vi "CSM-Logger-Thread(Event).vi"(4 "Log Limit":T1={"file size (in bytes)"=10000000, "file num"=2} {"file size (in bytes)" format="%.0p"}, 6 "Exit When All Module Exist? (F)":bool, 7 "Format String":string="%<%Y/%m/%d %H:%M:%S%3u>T", 8 "error in (no error)":errorcluster, 9 "WatchDogQ":refnum<queue>, 10 "GlobalLogFilter.lvclass":refnum<class "LogFilter.lvclass">, 11 "File Path (Use Dialog)":path) -> (0 "error out":errorcluster)   [LabVIEW 2017, in "CSM File Logger.lvlib"]
doc: "The thread VI originally used in the CSM - Start File Logger VI. This VI is now deprecated. Use the CSM-Logger-Thread VI.\n\n\n> [!NOTE] <b>CSM File Logger Implementation Principle</b>\n>\n> The CSM File Logger retrieves all execution records in the application via the CSM Global Log API and saves them to a specified text file for later analysis and error localization. The file format is a text file with the suffix `.csmlog`, which can be opened using text editing query tools such as Notepad."
uses:
  CSM File Logger.lvlib
  CSM File Logger Limit.ctl
  _Support/GlobalEvent/LogFilter/LogFilter.lvclass
  _Support/Typedef/_CSM_List Module Scope.ctl
  _Support/Typedef/_CSM_GlobalLog_MSG.ctl
  _Support/Typedef/_CSM_Response Source Message.ctl
  _Support/Typedef/_CSM_GlobalLog_MSG_TYPE.ctl
  Utility/_support/Periodic String Filter Level.ctl
  _Support/GlobalEvent/GEvt-Generate with Rule Check.vi
  AdvanceAPI/CSM - Convert Error to Argument.vi
  _Support/GlobalEvent/Cache-GEvt Filter Object.vi
  _Support/GlobalEvent/Cache-GEvt Refs.vi
  AdvanceAPI/CSM - Make String Arguments Safe.vi
  _Support/GlobalEvent/GEvt-Convert Filter Rules - v1.2.vi
  _Support/ChangeFlag/FlagInstance-GEvt Filter.vi
  _Support/ChangeFlag/FlagInstance-GEvt Refs.vi
  AdvanceAPI/CSM - Keywords.vi
  _Support/ChangeFlag/ChangeFlag-Read.vi
  _Support/GlobalEvent/LogFilter/SettingVIs/Set Periodic Log Filter.vi
  _Support/GlobalEvent/LogFilter/SettingVIs/Set CSM UserLog Filter.vi
  _Support/GlobalEvent/LogFilter/SettingVIs/Set CSM Broadcast Filter.vi
  _Support/GlobalEvent/LogFilter/SettingVIs/Set CSM StateType Filter.vi
  _Support/GlobalEvent/LogFilter/SettingVIs/Set Global StateType Filter.vi
  _Support/GlobalEvent/LogFilter/SettingVIs/Set CSM State Filter.vi
  _Support/GlobalEvent/LogFilter/SettingVIs/Set CSM LogType Filter.vi
  _Support/GlobalEvent/LogFilter/SettingVIs/Set Global UserLog Filter.vi
  _Support/GlobalEvent/LogFilter/SettingVIs/Set Global Broadcast Filter.vi
  _Support/GlobalEvent/LogFilter/SettingVIs/Set Global State Filter.vi
  _Support/GlobalEvent/LogFilter/SettingVIs/Set Global LogType Filter.vi
  _Support/GlobalEvent/LogFilter/SettingVIs/Set Global CSM Filter.vi
  _Support/GlobalEvent/FGV-GEvt Filter Rules(lvlibp).vi
  _Support/ChangeFlag/ChangeFlagDB.vi
  _Support/GlobalEvent/GEvt-Valid Subscribers.vi
  _Support/GlobalEvent/FGV-GlobalEventQueues(lvlibp).vi
  _Support/GlobalEvent/FGV-GlobalEventRef(lvlibp).vi
  Communicable State Machine.lvlib
panel:
  out "size (in bytes)":i64
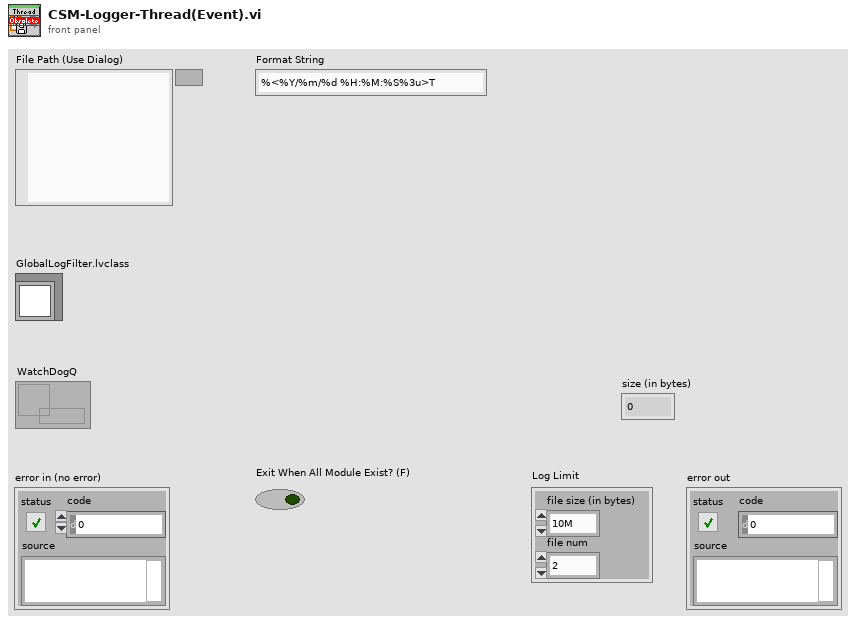
[diagram p1: front panel]
types:
  T1 = typedef "CSM File Logger.lvlib/CSM File Logger Limit.ctl" = cluster{"file size (in bytes)":i64, "file num":i32}
  T2 = typedef "Communicable State Machine.lvlib/_CSM_GlobalLog Filter Rules - v1.2.ctl" = cluster{"Global":cluster{"CSM":string[], "LogType":T3[], "State":string[], "StateType":T4[], "Broadcast":string[], "UserLog":string[]}, "CSM":cluster{"LogType":cluster{"CSM":string, "LogType":T3}[], "State":cluster{"CSM":string, "State":string}[], "StateType":cluster{"CSM":string, "LogType":T4}[], "Broadcast":cluster{"CSM":string, "Broadcast":string}[], "UserLog":cluster{"CSM":string, "UserLog":string}[]}, "PeriodicMessageFilter":cluster{"Enable":bool, "Threshold(#/s)":dbl, "CheckPeriod(s)":dbl}}
  T3 = typedef "Communicable State Machine.lvlib/_CSM_GlobalLog_MSG_TYPE.ctl" = enum16{"User Log", "State Change", "Status", "Interrupt", "Register", "Unregister", "Error Log", "Module Created", "Module Destroyed", "Async Message", "No-Rep Async Message", "Sync Message", "AsyncMsg Complete", "SyncMsg Complete"}
  T4 = typedef "Communicable State Machine.lvlib/_CSM_GlobalLog_STATE_TYPE.ctl" = enum16{"State - Internal State", "State - External Message", "State - Response", "State - Complete"}
  T5 = cluster{"Queue":path[], "folder":path, "name":string, "index":i32, "Log Limit":T1}
  T6 = typedef "Communicable State Machine.lvlib/_CSM_List Module Scope.ctl" = enum16{"Normal", "System Only", "All"}
  T7 = typedef "Communicable State Machine.lvlib/Periodic String Filter Level.ctl" = enum16{"normal", "L1", "L2", "L3", "L4"}
  T8 = typedef "Communicable State Machine.lvlib/_CSM_GlobalLog_MSG.ctl" = cluster{"Name (\"\" to Use UUID)":string, "Current State":string, "Arguments":string, "Source Message":T9, "Source Module":string, "Complete(T)/Start(F)":bool, "LogType":T3, "Time Stamp":timestamp}
  T9 = typedef "Communicable State Machine.lvlib/_CSM_Response Source Message.ctl" = cluster{"‘State":string, "’Arguments":string, "’Error":errorcluster}
  T10 = enum16{"open", "replace", "create", "open or create", "replace or create", "replace or create with confirmation"}
  T11 = cluster{"Major":u16, "Minor":u16, "Fix":u16, "Build":u16}
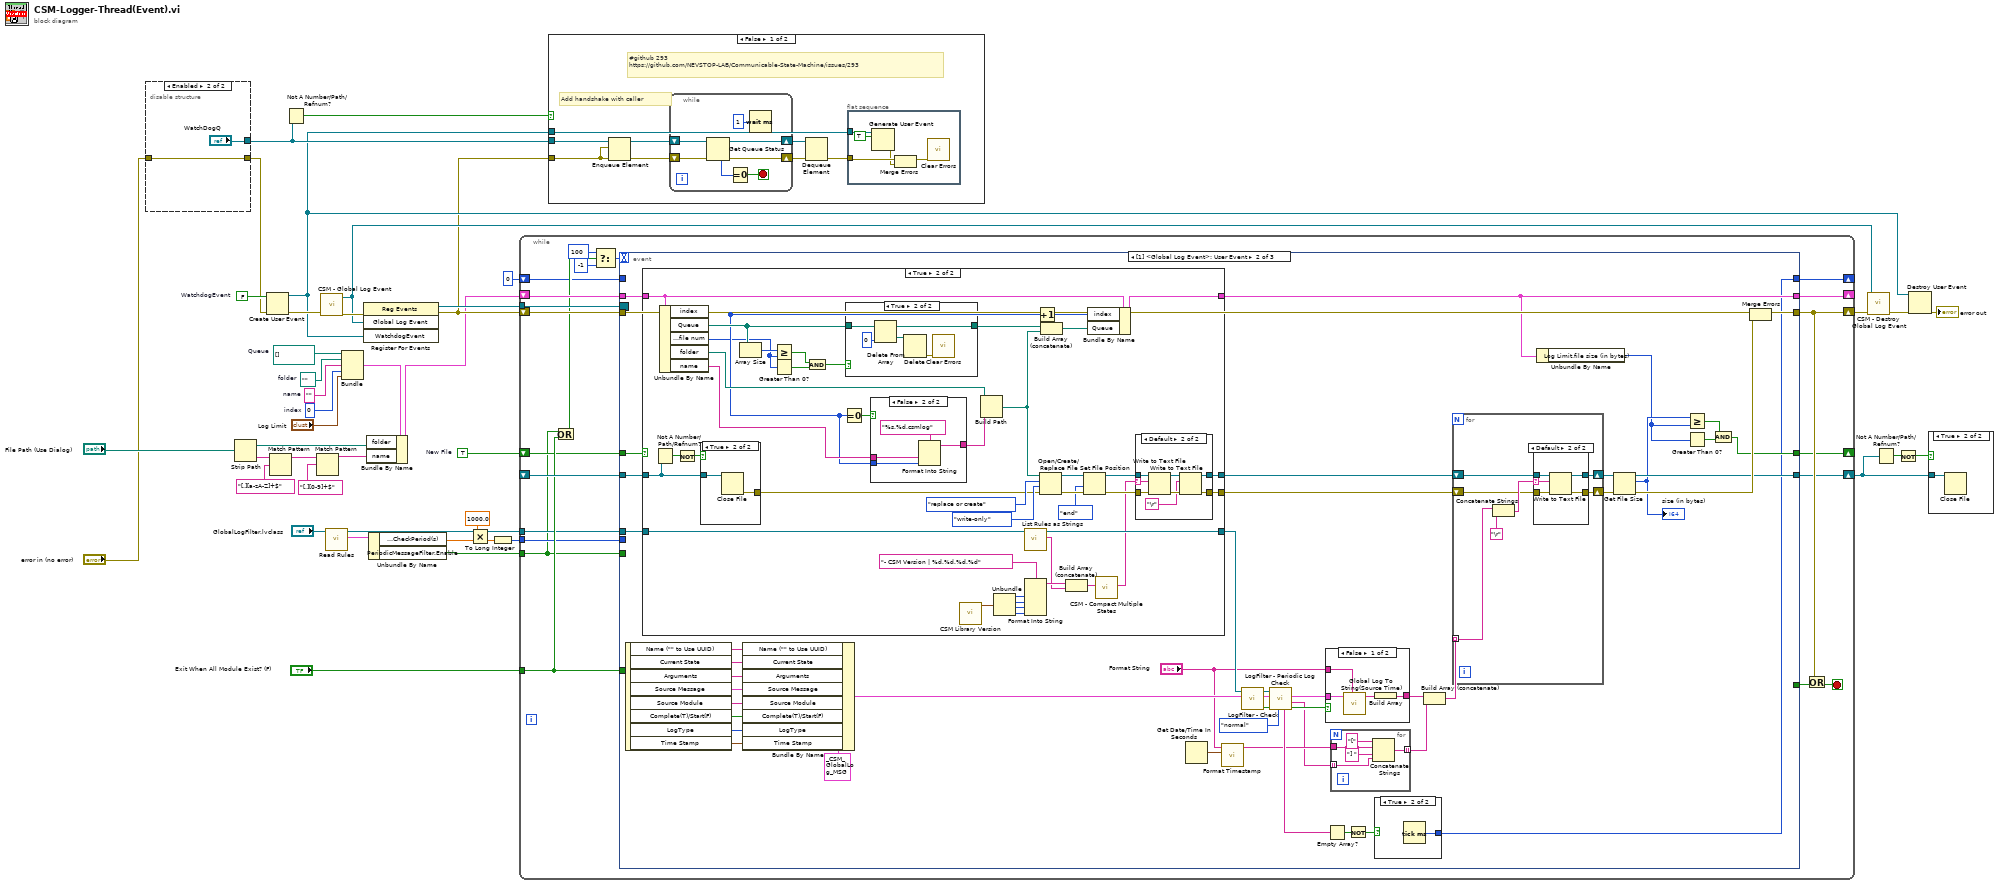
[diagram p0: block diagram]
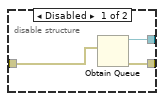
[diagram p2: hidden frame]
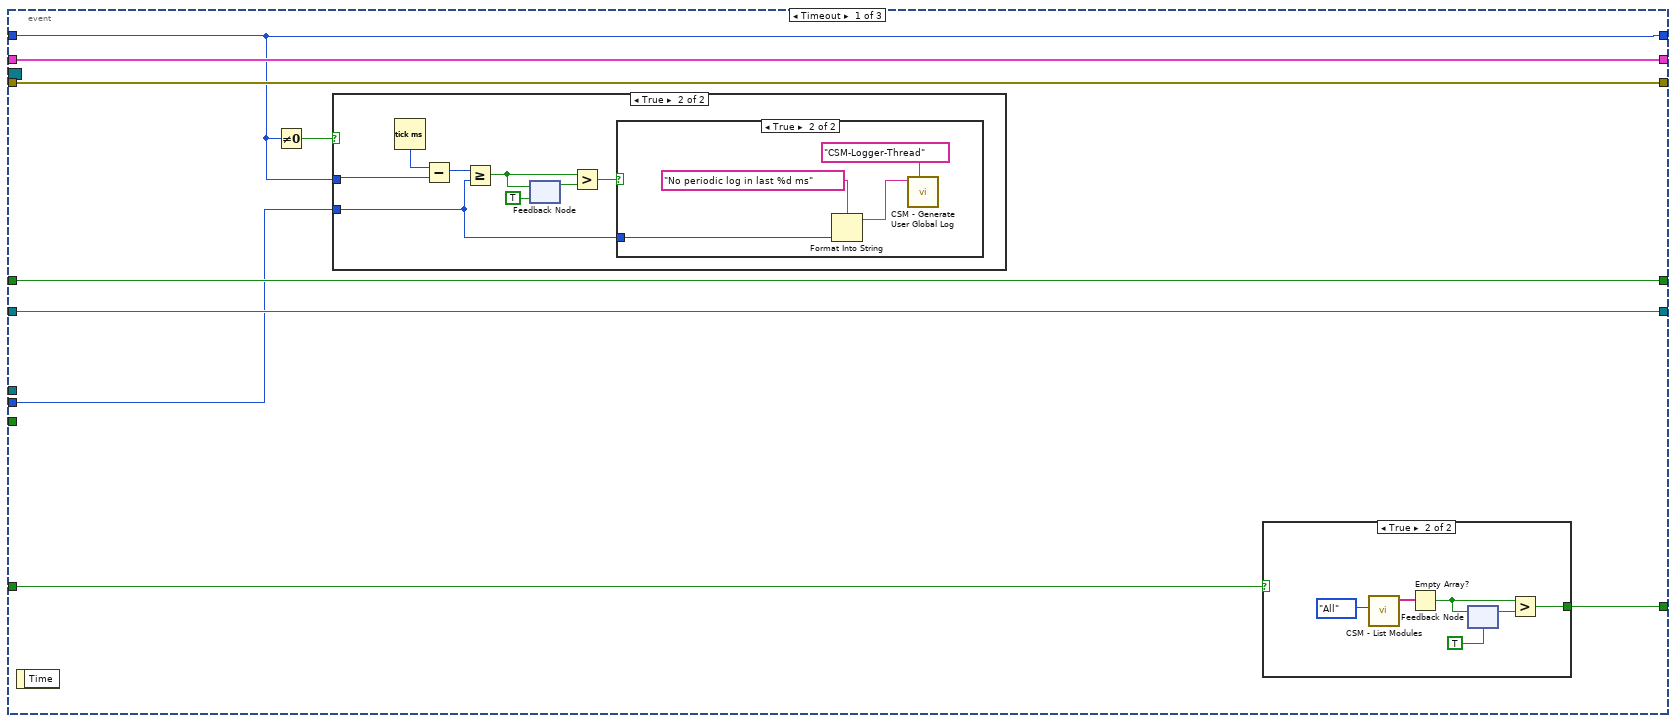
[diagram p5: hidden frame]
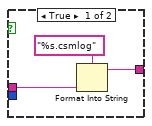
[diagram p14: hidden frame]
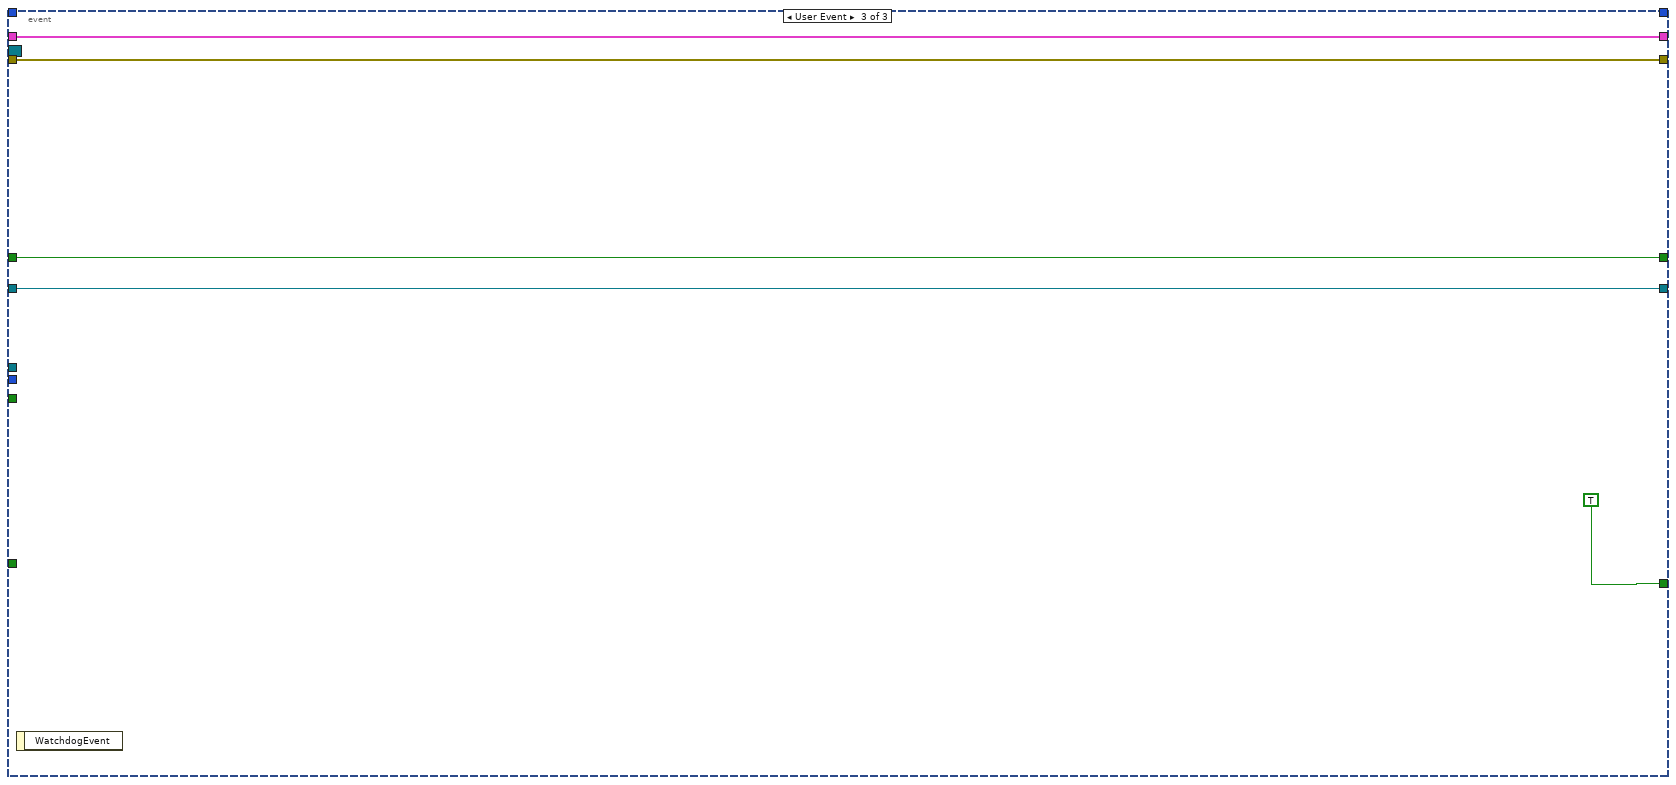
[diagram p17: hidden frame]
diagram:
  w19 = ""  # name
  w22 = 0  # index
  w23 = path ""  # folder
  w24 = path[] []  # Queue
  w27 = TRUE  # New File
  w36 = FALSE  # WatchdogEvent
  n1 = disable-structure shown="Enabled" {
    disable-tunnel: [w43 "WatchDogQ"] -> w38
    disable-tunnel: [w45 w46] -> w26
    disable-tunnel: "error in (no error)" -> [w44 w46]
    frame Disabled {
      n2 = Obtain Queue(element data type=w44) -> (queue out=w43:refnum<queue>, error out=w45:errorcluster)  [unwired: 4 in, 1 out]
    }
    frame Enabled {
    }
  }
  n3 = Strip Path(path="File Path (Use Dialog)") -> (stripped path=w12:path, name=w18:string)
  n4 = Create User Event(user event datatype=w36, error in=w26) -> (user event=w33:refnum<user-event>, error out=w35:errorcluster)
  n5 = Match Pattern(string=w18, regular expression="[.][a-zA-Z]+$") -> (before substring=w15:string)  [unwired: 1 in, 3 out]
  n6 = Not A Number/Path/Refnum?(number/path/refnum=w38) -> (NaN/Path/Refnum?=w37:bool)
  n7 = Match Pattern(string=w15, regular expression="[.][0-9]+$") -> (before substring=w13:string)  [unwired: 1 in, 3 out]
  n8 = call "CSM - Global Log Event.vi"("Error In"=w35) -> ("error out"=w40:errorcluster, "Global Log Event"=w39:refnum<user-event>)  [unwired: 9 in]
  n9 = call "Read Rules.vi"("LogFilter In"="GlobalLogFilter.lvclass") -> ("Rules"=w7:T2, "LogFilter Out"=w8:refnum<class "LogFilter.lvclass">)  [unwired: 8 in, 1 out]
  n10 = Bundle("Queue"=w24, "folder"=w23, "name"=w19, "index"=w22, "Log Limit"="Log Limit") -> (w20:T5)  [unwired: 1 in]
  n11 = register-events(error in=w40, w39, w33) -> (reference out=w42:refnum<event-registration>, error out=w25:errorcluster)  [unwired: 1 in]
  n12 = Bundle By Name(cluster=w20, "folder"=w12, "name"=w13) -> (w14:T5)
  n13 = Unbundle By Name(w7) -> ("PeriodicMessageFilter.CheckPeriod(s)"=w5:dbl, "PeriodicMessageFilter.Enable"=w6:bool)
  n14 = Multiply(x=1000.0, y=w5) -> (x*y=w4:dbl)
  n15 = To Long Integer(number=w4) -> (32bit integer=w2:i32)
  n16 = while {
    tunnel: w42 -> [w68]
    shift-right: [w65] -> w41
    shift-left: w25 -> [w67]
    shift-right: [w62] -> w30
    shift-left: _ -> [w63]
    tunnel: "Exit When All Module Exist? (F)" -> [w61]
    shift-right: [w57] -> _
    shift-left: w27 -> [w58]
    shift-right: [w55] -> _
    shift-left: w14 -> [w56]
    tunnel: w8 -> [w54]
    tunnel: w6 -> [w49]
    tunnel: w2 -> [w53]
    shift-right: [w52] -> _
    shift-left: u32 0 ("millisecond timer value") -> [w48]
    stop <- w66 stop-if-true
    n17 = Or(x=w49, y=w61) -> (x .or. y?=w50:bool)
    n18 = Select(t=100, s=w50, f=-1) -> (s? t:f=w59:i32)
    n19 = event shown="[1] <Global Log Event>: User Event" {
      selector: w68 -> [_ _ _]
      dyn-events: _ -> [_ _ _]
      timeout: w59 -> [_ _ _]
      tunnel: w67 -> [w77 w132 w240]
      tunnel: [w77 w131 w240] -> w65
      tunnel: [w75 _ TRUE ("rising edge")] -> w64
      tunnel: w63 -> [w76 w133 w239]
      tunnel: [w76 w124 w239] -> w62
      tunnel: w61 -> [w74 _ _]
      tunnel: w58 -> [w73 w128 w237]
      tunnel: [w73 w122 w237] -> w57
      tunnel: w56 -> [w72 w117 w236]
      tunnel: [w72 w118 w236] -> w55
      tunnel: w54 -> [_ w114 _]
      tunnel: w49 -> [_ _ _]
      tunnel: w53 -> [w69 _ _]
      tunnel: [w70 w102 _] -> w52
      tunnel: w48 -> [w70 _ _]
      event Timeout {
        n20 = event-data() -> ()  [unwired: 1 in, 1 out]
        n21 = Not Equal To 0?(x=w70) -> (x != 0?=w71:bool)
        n22 = case shown="True" w71 {
          tunnel: w70 -> [_ w84]
          tunnel: w69 -> [_ w79]
          frame False {
          }
          frame True {
            n23 = Tick Count (ms)() -> (millisecond timer value=w85:u32)
            n24 = Subtract(x=w85, y=w84) -> (x-y=w83:u32)
            n25 = Greater Or Equal?(x=w83, y=w79) -> (x >= y?=w82:bool)
            n26 = feedback-in #1(w82) -> ()
            n27 = feedback #1(TRUE) -> (w81:bool)
            n28 = Greater?(x=w82, y=w81) -> (0:w78:bool)
            n29 = case shown="True" w78 {
              tunnel: w79 -> [_ w86]
              frame False {
              }
              frame True {
                n30 = Format Into String(format string="No periodic log in last %d ms" ("Log"), w86) -> (resulting string=w87:string)  [unwired: 2 in, 1 out]
                n31 = call "CSM - Generate User Global Log.vi"("Place (\"\" to Use VI's Name)"="CSM-Logger-Thread" ("Place(\"\" to use VI's Name)"), "Log"=w87) -> ()  [unwired: 9 in, 1 out]
              }
            }
          }
        }
        n32 = case shown="True" w74 {
          tunnel: [_ w91] -> w75
          frame False {
          }
          frame True {
            n33 = call "CSM - List Modules.vi"("Scope (Normal)"=_CSM_List_Module_Scope."All" ("Mode")) -> ("Module Names"=w95:string[])  [unwired: 9 in, 1 out]
            n34 = Empty Array?(array=w95) -> (empty?=w94:bool)
            n35 = feedback #2(TRUE ("All?")) -> (w93:bool)
            n36 = feedback-in #2(w94) -> ()
            n37 = Greater?(x=w94, y=w93) -> (0:w91:bool)
          }
        }
      }
      event User Event {
        n38 = event-data() -> ("Name (\"\" to Use UUID)"=w141:string, "Current State"=w140:string, "Arguments"=w139:string, "Source Message"=w138:T9, "Source Module"=w137:string, "Complete(T)/Start(F)"=w136:bool, "LogType"=w135:T3, "Time Stamp"=w101:timestamp)  [unwired: 1 in]
        n39 = case shown="True" w128 {
          tunnel: w133 -> [w168 w208]
          tunnel: [_ w180] -> w130
          tunnel: [w168 w181] -> w129
          tunnel: [w167 w197] -> w118
          tunnel: w117 -> [w167 w199]
          tunnel: [w166 w179] -> w115
          tunnel: w114 -> [w166 w184]
          frame False {
          }
          frame True {
            n40 = Not A Number/Path/Refnum?(number/path/refnum=w208) -> (NaN/Path/Refnum?=w209:bool)
            n41 = Unbundle By Name(w199) -> ("index"=w189:i32, "Queue"=w200:path[], "Log Limit.file num"=w186:i32, "folder"=w193:path, "name"=w192:string)
            n42 = Not(x=w209) -> (.not. x?=w210:bool)
            n43 = case shown="True" w210 {
              tunnel: w208 -> [_ w235]
              tunnel: [_ w234] -> w202
              frame False {
              }
              frame True {
                n44 = Close File(refnum=w235) -> (error out=w234:errorcluster)  [unwired: 1 in, 1 out]
              }
            }
            n45 = Array Size(array=w200) -> (size(s)=w201:i32)
            n46 = Greater Or Equal?(x=w201, y=w186) -> (x >= y?=w188:bool)
            n47 = Greater Than 0?(x=w186) -> (x > 0?=w187:bool)
            n48 = And(x=w188, y=w187) -> (x .and. y?=w185:bool)
            n49 = Equal To 0?(x=w189) -> (x = 0?=w190:bool)
            n50 = case shown="True" w185 {
              tunnel: w200 -> [w228 w233]
              tunnel: [w228 w229] -> w198
              frame False {
              }
              frame True {
                n51 = Delete From Array(array=w233, index=0) -> (deleted portion=w231:path, array with subset deleted=w229:path[])  [unwired: 1 in]
                n52 = Delete(path (use dialog)=w231) -> (error out=w230:errorcluster)  [unwired: 4 in, 2 out]
                n53 = call <vilib>:"Clear Errors.vi"("error in (no error)"=w230) -> ()  [unwired: 5 in, 2 out]
              }
            }
            n54 = case shown="False" w190 {
              tunnel: [w222 w226] -> w194
              tunnel: w192 -> [w221 w225]
              tunnel: w189 -> [_ w224]
              frame True {
                n55 = Format Into String(format string="%s.csmlog", w221) -> (resulting string=w222:string)  [unwired: 2 in, 1 out]
              }
              frame False {
                n56 = Format Into String(format string="%s.%d.csmlog", w225, w224) -> (resulting string=w226:string)  [unwired: 2 in, 1 out]
              }
            }
            n57 = call "CSM Library Version.vi"() -> ("Min-Compatible Version"=w178:T11)  [unwired: 10 in, 1 out]
            n58 = Build Path(base path=w193, name or relative path=w194) -> (appended path=w191:path)
            n59 = Unbundle(w178) -> ("Major"=w174:u16, "Minor"=w175:u16, "Fix"=w176:u16, "Build"=w177:u16)
            n60 = call "List Rules as Strings.vi"("GlobalLogFilter In"=w184) -> ("Rule Strings"=w170:string[], "GlobalLogFilter Out"=w179:refnum<class "LogFilter.lvclass">)  [unwired: 8 in, 1 out]
            n61 = Format Into String(format string="- CSM Version | %d.%d.%d.%d" ("String to Prepend to Source (\"\")"), w174, w175, w176, w177) -> (resulting string=w172:string)  [unwired: 2 in, 1 out]
            n62 = Increment(x=w189) -> (x+1=w195:i32)
            n63 = Open/Create/Replace File(file path (use dialog)=w191, error in=w202, operation (0:open)=T10."replace or create", access (0:read/write)=enum16{"read/write", "read-only", "write-only"}."write-only") -> (refnum out=w207:refnum<file>, error out=w206:errorcluster)  [unwired: 2 in, 1 out]
            n64 = Build Array (concatenate)(w198, w191) -> (w196:path[])
            n65 = Build Array (concatenate)(w172, w170) -> (w171:string[])
            n66 = Set File Position(refnum=w207, from (0:start)=enum16{"start", "end", "current"}."end", error in=w206) -> (refnum out=w182:refnum<file>, error out=w183:errorcluster)  [unwired: 1 in]
            n67 = Bundle By Name(cluster=w199, "index"=w195, "Queue"=w196) -> (w197:T5)
            n68 = call "CSM - Compact Multiple States.vi"("Multiple States"=w171) -> ("States"=w169:string)  [unwired: 9 in]
            n69 = case shown="Default" w169 {
              selector: w169 -> [_ w220]
              tunnel: w183 -> [w211 w219]
              tunnel: w182 -> [w212 w218]
              tunnel: [w212 w215] -> w181
              tunnel: [w211 w214] -> w180
              frame "" {
              }
              frame Default {
                n70 = Write to Text File(file (use dialog)=w218, text=w220, error in=w219) -> (refnum out=w216:refnum<file>, error out=w217:errorcluster)  [unwired: 1 in, 1 out]
                n71 = Write to Text File(file (use dialog)=w216, text="\r", error in=w217) -> (refnum out=w215:refnum<file>, error out=w214:errorcluster)  [unwired: 1 in, 1 out]
              }
            }
          }
        }
        n72 = Bundle By Name(cluster=T8 {"Name (\"\" to Use UUID)"="", "Current State"="", "Arguments"="", "Source Message"={"‘State"="", "’Arguments"="", "’Error"={"status"=FALSE, "code"=0, "source"=""}}, "Source Module"="", "Complete(T)/Start(F)"=FALSE, "LogType"=enum."User Log", "Time Stamp"=timestamp(0 s since 1904-01-01)} ("Cross CSM Data"), "Name (\"\" to Use UUID)"=w141, "Current State"=w140, "Arguments"=w139, "Source Message"=w138, "Source Module"=w137, "Complete(T)/Start(F)"=w136, "LogType"=w135, "Time Stamp"=w101) -> (w116:T8)
        n73 = Get Date/Time In Seconds() -> (seconds since 1Jan1904=w108:timestamp)
        n74 = call "Format Timestamp.vi"("Timestamp"=w108, "Format String"="Format String") -> ("String"=w100:string)  [unwired: 9 in]
        n75 = call "LogFilter - Check.vi"("Cross CSM Data In"=w116, "GlobalLogFilter In"=w115) -> ("Matched? (Dup)"=w110:bool, "Cross CSM Data Out"=w111:T8, "GlobalLogFilter.lvclass (Dup)"=w113:refnum<class "LogFilter.lvclass">)  [unwired: 7 in]
        n76 = call "LogFilter - Periodic Log Check.vi"("Level (Normal)"=Periodic_String_Filter_Level."normal" ("Level(Normal)"), "Matched Previous?"=w110, "Cross CSM Data In"=w111, "GlobalLogFilter In"=w113) -> ("Matched? (Dup)"=w107:bool, "Additional Info"=w99:string[], "Cross CSM Data Out"=w112:T8, "Filtered Status"=w105:string[])  [unwired: 3 in, 1 out]
        n77 = case shown="False" w107 {
          tunnel: w112 -> [w165 _]
          tunnel: [w163 _] -> w109
          tunnel: "Format String" -> [w162 _]
          frame False {
            n78 = call "Global Log To String(Source Time).vi"("Format String"=w162, "Log"=w165) -> ("Log String"=w164:string)  [unwired: 8 in]
            n79 = Build Array(w164) -> (w163:string[])
          }
          frame True {
          }
        }
        n80 = Empty Array?(array=w105) -> (empty?=w104:bool)
        n81 = for {
          tunnel: w100 -> [w144]
          tunnel: w99 -> [w143] mode=indexing
          tunnel: [w142] -> w98 mode=indexing
          n82 = Concatenate Strings("[" ("string"), w144, "] " ("string"), w143) -> (w142:string)
        }
        n83 = Not(x=w104) -> (.not. x?=w103:bool)
        n84 = case shown="True" w103 {
          tunnel: [_ w147] -> w102
          frame False {
          }
          frame True {
            n85 = Tick Count (ms)() -> (millisecond timer value=w147:u32)
          }
        }
        n86 = Build Array (concatenate)(w109, w98) -> (w106:string[])
        n87 = for {
          tunnel: w106 -> [w148] mode=indexing
          shift-right: [w150] -> w126
          shift-left: w130 -> [w153]
          shift-right: [w151] -> w127
          shift-left: w129 -> [w152]
          n88 = Concatenate Strings(w148, "\r") -> (w154:string)
          n89 = case shown="Default" w154 {
            selector: w154 -> [_ w161]
            tunnel: w153 -> [w155 w160]
            tunnel: w152 -> [w156 w159]
            tunnel: [w156 w158] -> w151
            tunnel: [w155 w157] -> w150
            frame "" {
            }
            frame Default {
              n90 = Write to Text File(file (use dialog)=w159, text=w161, error in=w160) -> (refnum out=w158:refnum<file>, error out=w157:errorcluster)  [unwired: 1 in, 1 out]
            }
          }
        }
        n91 = Unbundle By Name(w118) -> ("Log Limit.file size (in bytes)"=w119:i64)
        n92 = Get File Size(file=w127, error in=w126) -> (refnum out=w124:refnum<file>, size (in bytes)=w123:i64, 0:w125:errorcluster)
        "size (in bytes)" <- w123
        n93 = Greater Or Equal?(x=w123, y=w119) -> (x >= y?=w121:bool)
        n94 = Greater Than 0?(x=w119) -> (x > 0?=w120:bool)
        n95 = And(x=w121, y=w120) -> (x .and. y?=w122:bool)
        n96 = Merge Errors(w132, w125) -> (w131:errorcluster)
      }
      event User Event {
        n97 = event-data() -> ()  [unwired: 1 in, 1 out]
      }
    }
    n98 = Or(x=w65, y=w64) -> (x .or. y?=w66:bool)
  }
  n99 = case shown="False" w37 {
    tunnel: w38 -> [w246 _]
    tunnel: w33 -> [w247 _]
    tunnel: w25 -> [w241 _]
    frame False {
      # "#github 293 \nhttps://github.com/NEVSTOP-LAB/Communicable-State-Machine/issues/293"
      # "Add handshake with caller"
      n100 = Enqueue Element(queue=w246, element=w241, error in (no error)=w241) -> (queue out=w245:refnum<queue>, error out=w243:errorcluster)  [unwired: 1 in, 1 out]
      n101 = while {
        shift-right: [w254] -> w244
        shift-left: w245 -> [w255]
        shift-right: [w252] -> w242
        shift-left: w243 -> [w253]
        stop <- w250 stop-if-true
        n102 = Get Queue Status(queue=w255, error in (no error)=w253) -> (queue out=w254:refnum<queue>, error out=w252:errorcluster, # elements in queue=w251:i32)  [unwired: 1 in, 5 out]
        n103 = Equal To 0?(x=w251) -> (x = 0?=w250:bool)
        n104 = Wait (ms)(milliseconds to wait=u32 1) -> ()  [unwired: 1 out]
      }
      n105 = Dequeue Element(queue=w244, error in (no error)=w242) -> (error out=w248:errorcluster)  [unwired: 1 in, 3 out]
      n106 = flat-sequence {
        tunnel: w248 -> [w259]
        tunnel: w247 -> [w260]
        frame #0 {
          n107 = Generate User Event(user event=w260, event data cluster=TRUE ("event data")) -> (error out=w257:errorcluster)  [unwired: 2 in, 1 out]
          n108 = Merge Errors(w259, w257) -> (w258:errorcluster)
          n109 = call <vilib>:"Clear Errors.vi"("error in (no error)"=w258) -> ()  [unwired: 5 in, 2 out]
        }
      }
    }
    frame True {
    }
  }
  n110 = call "CSM - Destroy Global Log Event.vi"("Error In"=w41, "CSM Global Log Event"=w39) -> ("error out"=w34:errorcluster)  [unwired: 9 in]
  n111 = Not A Number/Path/Refnum?(number/path/refnum=w30) -> (NaN/Path/Refnum?=w31:bool)
  n112 = Not(x=w31) -> (.not. x?=w29:bool)
  n113 = Destroy User Event(user event=w33, error in=w34) -> (error out=→"error out":errorcluster)
  n114 = case shown="True" w29 {
    tunnel: w30 -> [_ w261]
    frame False {
    }
    frame True {
      n115 = Close File(refnum=w261) -> ()  [unwired: 1 in, 2 out]
    }
  }
